vi "AutoToggle.vi"(8 "error in":T1) -> ()   [LabVIEW 2014]
uses:
  ErrorOut.ctl
  <vilib>/Rock Robotics/Network Tables/SD Write Boolean.vi
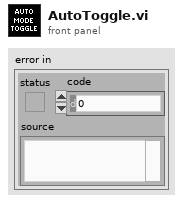
[diagram p1: front panel]
types:
  T1 = typedef "ErrorOut.ctl" = errorcluster
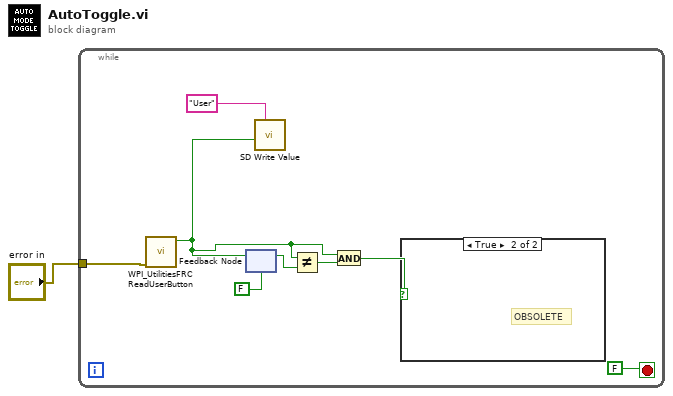
[diagram p0: block diagram]
diagram:
  n1 = while {
    tunnel: "error in" -> [w3]
    stop <- FALSE stop-if-true
    n2 = call <vilib>:"WPI_UtilitiesFRC ReadUserButton.vi"("error in"=w3) -> ("User Button"=w2:bool)  [unwired: 9 in, 1 out]
    n3 = feedback-in #1(w2) -> ()
    n4 = feedback #1(FALSE) -> (w4:bool)
    n5 = call-poly <vilib>:"SD Write Value.vi"("Boolean"=w2, "Name"="User") -> ()  [unwired: 8 in, 2 out]
    n6 = Not Equal?(x=w2, y=w4) -> (x != y?=w5:bool)
    n7 = And(x=w2, y=w5) -> (x .and. y?=w7:bool)
    n8 = case shown="True" w7 {
      frame False {
      }
      frame True {
        # "OBSOLETE"
      }
    }
  }
